vi "Long signal time plot data.vi"(8 "Time A Table Tag":string[](array[string]), 9 "Time Profile Table":string[][](table) caption="Time Table", 10 "CP A Tag AZ":string[](array[string]), 11 "CP Profile Table for plot":string[][](table) caption="CP Profile Table for Plot") -> (0 "Time A Table AZ":string[](array[string]), 3 "L Time Profile Table for plot":string[][](table) caption="L Time Table for plot")   [LabVIEW 2018]
panel:
  out "CP T IDX End [n]":string[](array[string])
  out "CP T IDX Start [n]":string[](array[string])
  out "サイズ":i32
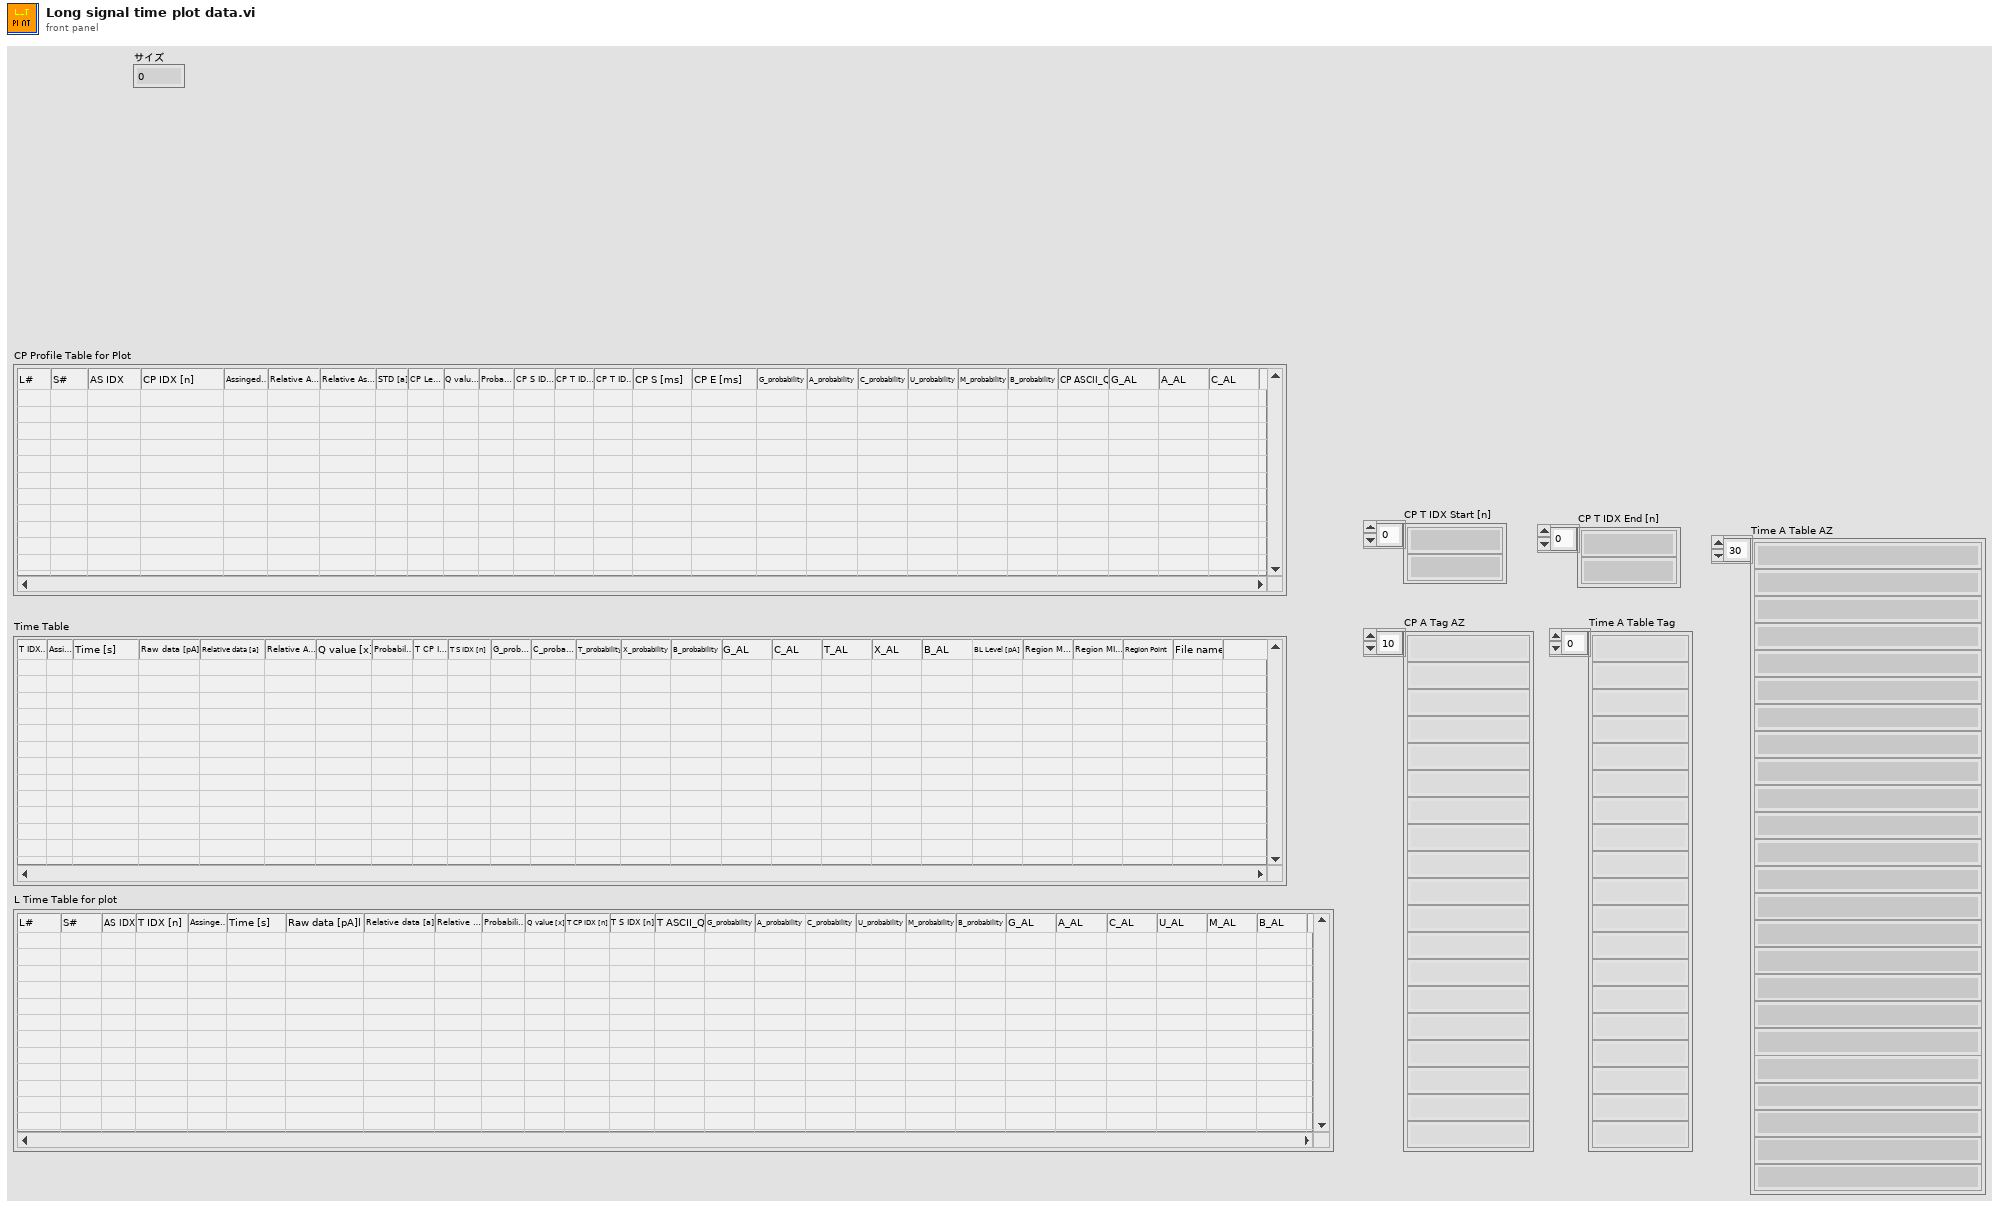
[diagram p1: front panel]
types:
  T1 = cluster{"CP T IDX Start [n]":string[], "CP T IDX End [n]":string[], "AS IDX":string[], "L#":string[], "S#":string[], "S/N ratio":string[], "Signal Intensity [pA]":string[], "BLX Level [pA]":string[], "Mx Intensity level [pA]":string[], "MS_IDX":string[], "Direction":string[], "Assinged Sequence":string[], "Mx Right Read Seq":string[], "Mx Right No":string[], "M_RRead_Seq":string[], "M_MxRight_No":string[]}
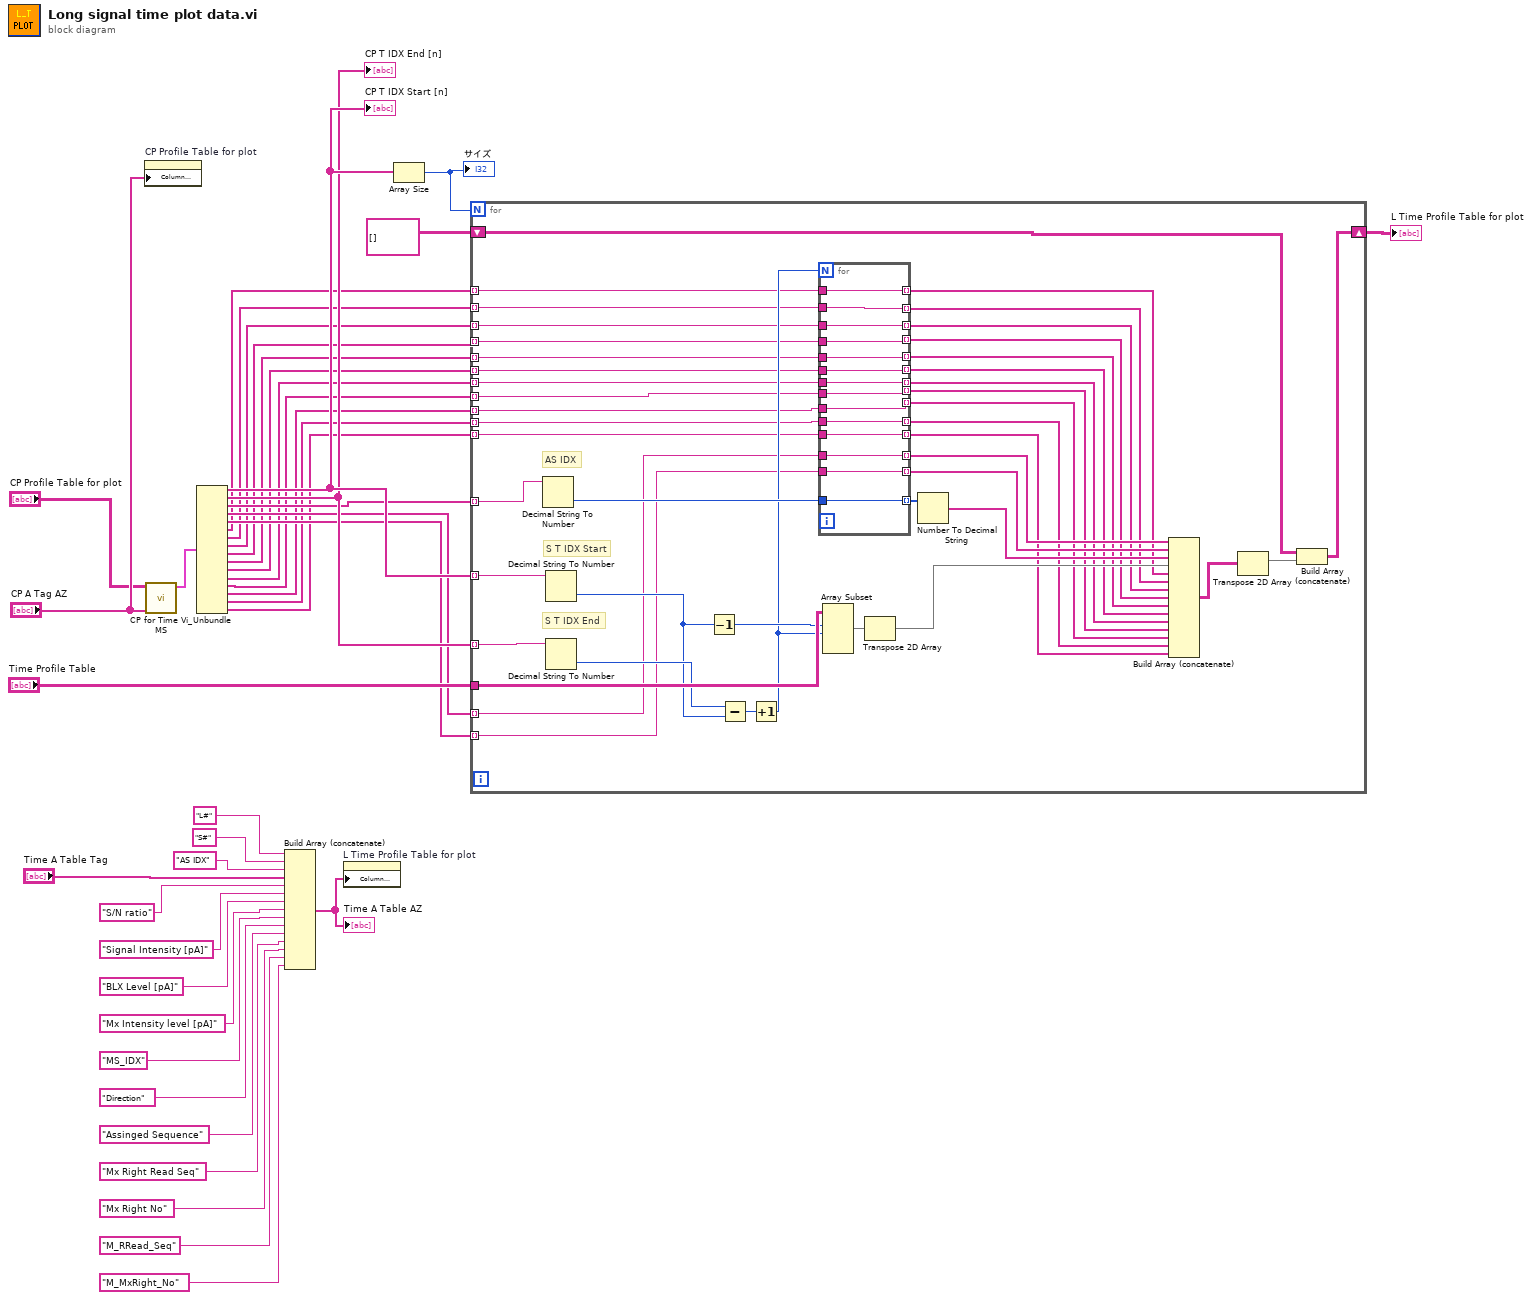
[diagram p0: block diagram]
diagram:
  n1 = property on="CP Profile Table for plot" class="Tbl (strict)"("Column Headers[]"="CP A Tag AZ") -> ()  [unwired: 2 in, 2 out]
  n2 = call "CP for Time Vi_MS.vi"("CP A Tag"="CP A Tag AZ", "CP Profile Table for All Seql"="CP Profile Table for plot") -> ("CPIDXZ"=w28:T1)  [unwired: 9 in]
  n3 = Unbundle(w28) -> ("CP T IDX Start [n]"=w27:string[], "CP T IDX End [n]"=w26:string[], "AS IDX"=w25:string[], "L#"=w24:string[], "S#"=w23:string[], "S/N ratio"=w11:string[], "Signal Intensity [pA]"=w10:string[], "BLX Level [pA]"=w9:string[], "Mx Intensity level [pA]"=w8:string[], "MS_IDX"=w7:string[], "Direction"=w6:string[], "Assinged Sequence"=w5:string[], "Mx Right Read Seq"=w4:string[], "Mx Right No"=w3:string[], "M_RRead_Seq"=w2:string[], "M_MxRight_No"=w1:string[])
  "CP T IDX Start [n]" <- w27
  "CP T IDX End [n]" <- w26
  n4 = Build Array (concatenate)("L#" ("y"), "S#" ("y"), "AS IDX" ("y"), "Time A Table Tag", "S/N ratio", "Signal Intensity [pA]", "BLX Level [pA]", "Mx Intensity level [pA]", "MS_IDX", "Direction", "Assinged Sequence", "Mx Right Read Seq", "Mx Right No", "M_RRead_Seq", "M_MxRight_No") -> (w33:string[])
  "Time A Table AZ" <- w33
  n5 = property on="L Time Profile Table for plot" class="Tbl (strict)"("Column Headers[]"=w33) -> ()  [unwired: 2 in, 2 out]
  n6 = Array Size(array=w27) -> (size(s)=w39:i32)
  "サイズ" <- w39
  n7 = for {
    N: w39 -> [_]
    tunnel: w27 -> [w83] mode=indexing
    tunnel: w26 -> [w82] mode=indexing
    tunnel: "Time Profile Table" -> [w81]
    tunnel: w25 -> [w76] mode=indexing
    shift-right: [w68] -> w36
    shift-left: string[][] [] -> [w69]
    tunnel: w24 -> [w65] mode=indexing
    tunnel: w23 -> [w64] mode=indexing
    tunnel: w11 -> [w61] mode=indexing
    tunnel: w10 -> [w60] mode=indexing
    tunnel: w9 -> [w59] mode=indexing
    tunnel: w8 -> [w58] mode=indexing
    tunnel: w7 -> [w57] mode=indexing
    tunnel: w6 -> [w56] mode=indexing
    tunnel: w5 -> [w55] mode=indexing
    tunnel: w4 -> [w54] mode=indexing
    tunnel: w3 -> [w53] mode=indexing
    tunnel: w2 -> [w52] mode=indexing
    tunnel: w1 -> [w51] mode=indexing
    # "AS IDX"
    # "S T IDX End"
    # "S T IDX Start"
    n8 = Decimal String To Number(string=w76) -> (number=w73:i32)  [unwired: 2 in, 1 out]
    n9 = Decimal String To Number(string=w83) -> (number=w78:i32)  [unwired: 2 in, 1 out]
    n10 = Decimal String To Number(string=w82) -> (number=w79:i32)  [unwired: 2 in, 1 out]
    n11 = Decrement(x=w78) -> (x-1=w80:i32)
    n12 = Subtract(x=w79, y=w78) -> (x-y=w77:i32)
    n13 = Increment(x=w77) -> (x+1=w70:i32)
    n14 = for {
      N: w70 -> [_]
      tunnel: w73 -> [w97]
      tunnel: [w97] -> w72 mode=indexing
      tunnel: w65 -> [w96]
      tunnel: w64 -> [w95]
      tunnel: [w96] -> w63 mode=indexing
      tunnel: [w95] -> w62 mode=indexing
      tunnel: w61 -> [w94]
      tunnel: w60 -> [w93]
      tunnel: w59 -> [w92]
      tunnel: w58 -> [w91]
      tunnel: w57 -> [w90]
      tunnel: w56 -> [w89]
      tunnel: w55 -> [w88]
      tunnel: w54 -> [w87]
      tunnel: w53 -> [w86]
      tunnel: w52 -> [w85]
      tunnel: w51 -> [w84]
      tunnel: [w94] -> w50 mode=indexing
      tunnel: [w93] -> w49 mode=indexing
      tunnel: [w92] -> w48 mode=indexing
      tunnel: [w91] -> w47 mode=indexing
      tunnel: [w90] -> w46 mode=indexing
      tunnel: [w89] -> w45 mode=indexing
      tunnel: [w88] -> w44 mode=indexing
      tunnel: [w87] -> w43 mode=indexing
      tunnel: [w86] -> w42 mode=indexing
      tunnel: [w85] -> w40 mode=indexing
      tunnel: [w84] -> w41 mode=indexing
    }
    n15 = Array Subset(array=w81, index (row)=w80, length (row)=w70) -> (w75:string[][])  [unwired: 2 in]
    n16 = Transpose 2D Array(2D array=w75) -> (transposed array=w74:string[][])
    n17 = Number To Decimal String(number=w72) -> (decimal integer string=w71:string[])  [unwired: 1 in]
    n18 = Build Array (concatenate)(w63, w62, w71, w74, w50, w49, w48, w47, w46, w45, w44, w43, w42, w40, w41) -> (w67:string[][])
    n19 = Transpose 2D Array(2D array=w67) -> (transposed array=w66:string[][])
    n20 = Build Array (concatenate)(w69, w66) -> (w68:string[][])
  }
  "L Time Profile Table for plot" <- w36
